vi "NetworkUDP_Recieve.vi"(8 "error in (no error)":errorcluster, 9 "timeout ms (25000)":i32=25000, 10 "IP4 address":u32, 11 "receiver port":u16=5801) -> (0 "error out":errorcluster, 1 "UDP Network Connection out":refnum<k16>, 2 "ConsecErrCount":i32, 3 "data out":string, 4 "SenderAddress":u32, 6 "SenderSrcPort":u16)   [LabVIEW 2019, in "Trajectory_Library.lvlib"]
doc: "Listen for and read a packet of data from the network using the UDP protocol. This routine can listen for a single computer or listen for any senders on the subnet. \n\nThis subVI does not return to the caller until either data has been received or a timeout has occured. Suggest putting this function in a separate loop to avoid issues slowing down other code.\n\nInputs:\n -- Receiver Port -- UInt16 -- UDP port number used for listening. Only data sent to this port will be returned. (Optional. Default: 5801)\n -- IP4 Address -- UInt32 -- The IP address of the computer expected to send data. If this value is 0, then then data will be returned for any sender. Use the standard TCP/IP LabVIEW functions to convert a standard IP4 address in the form of 123.123.123.123 to an unsigned integer for this input. (Optional. Default: 0) \n -- Timeout ms -- Int32 -- Timeout value in milliseconds. (Optional. Default: 25000 )\n -- Error in -- Error cluster -- Propagated error cluster. (Optional. Default: no error)\n\nOutputs:\n -- data out -- string -- Last data message sent to the specified port number.\n -- Consec Err -- Int32 -- Counter indicating the number of consecutive errors that have occured.\n -- UDP Network Connection -- UDP Connection Reference -- Reference to the UDP network connection. When finished with communication, the connection should be closed.\n -- SenderAddress -- Sender IP address (UInt32)\n -- SenderSrcPort -- Sender source port number\n -- Error out -- Error cluster -- Current propagated error cluster."
uses:
  Trajectory_Library.lvlib
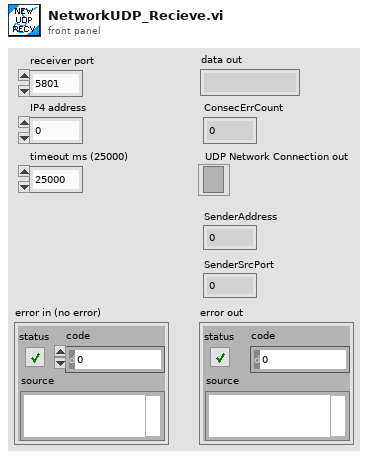
[diagram p1: front panel]
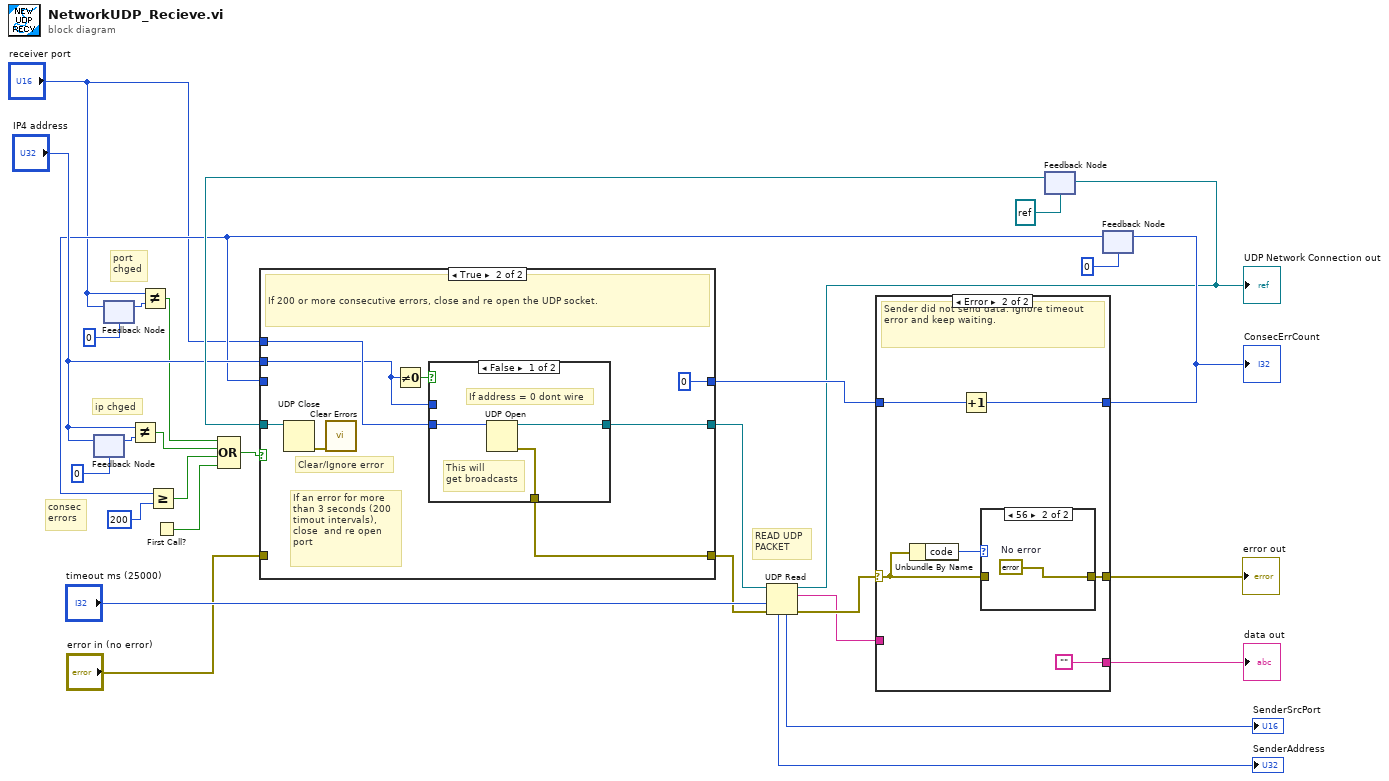
[diagram p0: block diagram]
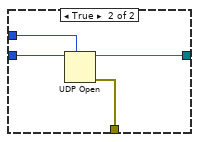
[diagram p3: hidden frame]
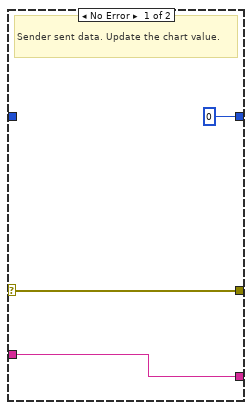
[diagram p4: hidden frame]
diagram:
  # "consec\nerrors"
  # "ip chged"
  # "port\nchged"
  # "READ UDP\nPACKET"
  n1 = feedback-in #1("IP4 address") -> ()
  n2 = feedback #1(u32 0 ("IP4 address")) -> (w16:u32)
  n3 = feedback #2(u16 0 ("receiver port")) -> (w5:u16)
  n4 = feedback-in #2("receiver port") -> ()
  n5 = Not Equal?(x="IP4 address", y=w16) -> (x != y?=w13:bool)
  n6 = Not Equal?(x="receiver port", y=w5) -> (x != y?=w2:bool)
  n7 = First Call?() -> (First Call?: T/F=w10:bool)
  n8 = feedback #3(refnum<k16> refnum ("port")) -> (w23:refnum<k16>)
  n9 = feedback #4(0) -> (w12:i32)
  n10 = Greater Or Equal?(x=w12, y=200) -> (x >= y?=w11:bool)
  n11 = Compound Arithmetic op=OR(w2, w13, w11, w10) -> (w14:bool)
  n12 = case shown="True" w14 {
    tunnel: w12 -> [w32 _]
    tunnel: [w32 0] -> w19
    tunnel: w23 -> [w31 w40]
    tunnel: [w31 w39] -> w22
    tunnel: "error in (no error)" -> [w30 _]
    tunnel: [w30 w38] -> w20
    tunnel: "receiver port" -> [_ w36]
    tunnel: "IP4 address" -> [_ w34]
    frame False {
      # "Not greater than 200 consecutive errors"
    }
    frame True {
      # "Clear/Ignore error"
      # "If an error for more\nthan 3 seconds (200 \ntimout intervals), \nclose  and re open \nport"
      # "If 200 or more consecutive errors, close and re open the UDP socket."
      n13 = UDP Close(connection ID=w40) -> (error out=w33:errorcluster)  [unwired: 1 in, 1 out]
      n14 = call <vilib>:"Clear Errors.vi"("error in (no error)"=w33) -> ()  [unwired: 5 in, 2 out]
      n15 = Not Equal To 0?(x=w34) -> (x != 0?=w35:bool)
      n16 = case shown="False" w35 {
        tunnel: [w42 w47] -> w39
        tunnel: [w43 w46] -> w38
        tunnel: w36 -> [w41 w45]
        tunnel: w34 -> [_ w44]
        frame False {
          # "This will\nget broadcasts"
          # "If address = 0 dont wire"
          n17 = UDP Open(11:w41) -> (port=w42:refnum<k16>, 0:w43:errorcluster)  [unwired: 4 in, 1 out]
        }
        frame True {
          n18 = UDP Open(7:w44, 11:w45) -> (port=w47:refnum<k16>, 0:w46:errorcluster)  [unwired: 3 in, 1 out]
        }
      }
    }
  }
  n19 = UDP Read(connection ID=w22, timeout ms (25000)="timeout ms (25000)", 8:w20) -> (data out=w27:string, error out=w28:errorcluster, 3:w7:refnum<k16>, 4:→"SenderSrcPort":u16, 6:→"SenderAddress":u32)  [unwired: 1 out]
  "UDP Network Connection out" <- w7
  n20 = case shown="Error" w28 {
    selector: w28 -> [w50 w55]
    tunnel: w27 -> [w49 _]
    tunnel: [w50 w54] -> w6
    tunnel: w19 -> [_ w53]
    tunnel: [w49 ""] -> w9
    tunnel: [0 w52] -> w8
    frame No Error {
      (unwired) 0
      # "Sender sent data. Update the chart value."
    }
    frame Error {
      # "Sender did not send data. Ignore timeout error and keep waiting."
      n21 = Unbundle By Name(w55) -> ("code"=w56:i32)
      n22 = Increment(x=w53) -> (x+1=w52:i32)
      n23 = case shown="56" w56 {
        tunnel: w55 -> [w57 _]
        tunnel: [w57 w58] -> w54
        frame Default {
        }
        frame 56 {
          w58 = errorcluster {"status"=FALSE, "code"=0, "source"=""}  # No error
        }
      }
    }
  }
  "error out" <- w6
  "ConsecErrCount" <- w8
  "data out" <- w9
  n24 = feedback-in #3(w7) -> ()
  n25 = feedback-in #4(w8) -> ()
